vi "Lamps_global.vi"() -> ()   [LabVIEW 2025]
panel:
  in  "Headers":string[](array[string])
  in  "LAMP COMPONENT":u16(ring) items=["", "HEAD LAMP", "TAIL LAMP", "INDICATORS", "OTHER LAMPS"]
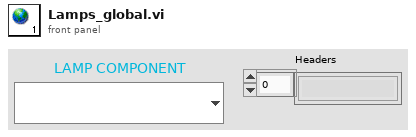
[diagram p1: front panel]
diagram:
